vi "Connect OPC UA.vi"(8 "error in":errorcluster, 9 "Trial Number":i32=3, 10 "URL":string="opc.tcp://DESKTOP-T6QR0HI:4991/LunarTester", 11 "Abstract":refnum<class "Abstract.lvclass">) -> (0 "error out":errorcluster={"status"=TRUE, "code"=97, "source"="Unknown System Error in TestStand - Initialize Termination Monitor.vi->Login Progress.vi"}, 3 "Abstract out":refnum<class "Abstract.lvclass">)   [LabVIEW 2025, in "Abstract.lvclass"]
uses:
  Abstract.lvclass
  Abstract.lvclass/Abstract.ctl
  Write OPC UA Ref.vi
  <vilib>/Utility/error.llb/Trim Whitespace One-Sided.vi
  <vilib>/OPCUA/client/Connect2.vi
  <vilib>/OPCUA/NI OPC UA Client.lvlib
panel:
  out "Connecting...":i32
  out "connected":bool
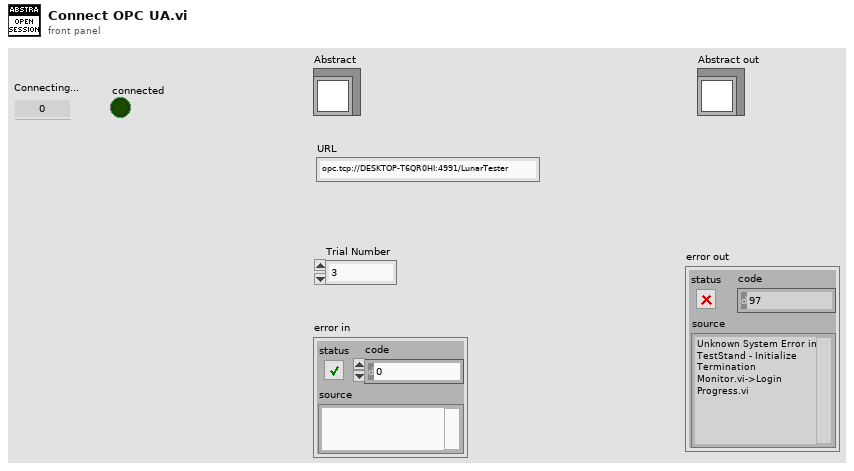
[diagram p1: front panel]
types:
  T1 = typedef "OPC UA Client Refnum.ctl" = refnum<k21>
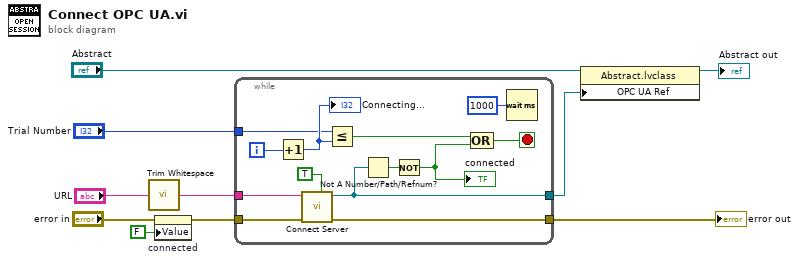
[diagram p0: block diagram]
diagram:
  n1 = call <vilib>:"Trim Whitespace.vi"("string"="URL") -> ("trimmed string"=w1:string)  [unwired: 1 in]
  n2 = property on="connected" class="Bool (strict)"(error in="error in", "Value"=FALSE ("stop")) -> (error out=w2:errorcluster)  [unwired: 1 in, 1 out]
  n3 = while {
    tunnel: w1 -> [w17]
    tunnel: "Trial Number" -> [w18]
    tunnel: [w14] -> w3
    tunnel: w2 -> [w16]
    tunnel: [w13] -> w8
    i -> [w23]
    stop <- w19 stop-if-true
    n4 = Increment(x=w23) -> (x+1=w22:i32)
    "Connecting..." <- w22
    n5 = call-poly <vilib>:"Connect Server.vi"("trust any server (F)"=TRUE, "error in (no error)"=w16, "server endpoint URL"=w17) -> ("error out"=w13:errorcluster, "OPC UA client refnum out"=w14:T1)  [unwired: 6 in, 1 out]
    n6 = Less Or Equal?(x=w18, y=w22) -> (x <= y?=w20:bool)
    n7 = Not A Number/Path/Refnum?(number/path/refnum=w14) -> (NaN/Path/Refnum?=w21:bool)
    n8 = Not(x=w21) -> (.not. x?=w11:bool)
    "connected" <- w11
    n9 = Compound Arithmetic op=OR(w20, w11) -> (w19:bool)
    n10 = Wait (ms)(milliseconds to wait=u32 1000) -> ()  [unwired: 1 out]
  }
  "error out" <- w8
  n11 = property class="Abstract.lvclass"(reference="Abstract", "OPC UA Ref"=w3) -> (reference out=→"Abstract out":refnum<class "Abstract.lvclass">)  [unwired: 1 in, 1 out]
